vi "Main Page.vi"(8 "error in":errorcluster, 11 "Node Ptr":T1 format="%.0x") -> (0 "error out":errorcluster)   [LabVIEW 2020, in "AIM ARINC 429 System Explorer.lvlib" / "Implementation.lvlib"]
uses:
  Implementation.lvlib
  <vilib>/NI VeriStand/Custom Device API/Custom Device API.lvlib
  Scripting/AIM/AIM ARINC 429 Scripting.lvlib
  <vilib>/NI VeriStand/Custom Device API/Custom Device Item Ref.ctl
panel:
  in  "Coupling Mode":enum32{"External", "Dual", "Internal"}(ring)
  in  "Async Rx Execution":bool
  in  "Decimation":i32=1 min=1
  in  "General Header":cluster{"Section Name":string}={"Section Name"="AIM ARINC 429 - Main"}
  in  "PXI Slot Number":u8=1
  in  "SHDocVw.IWebBrowser":refnum<k7>(container)
  in  "Description":string
  in  "Name":string
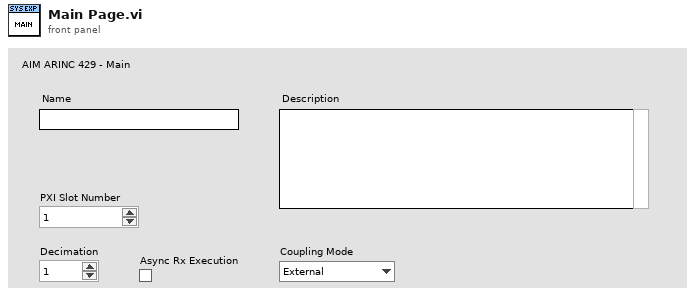
[diagram p1: front panel]
types:
  T1 = typedef "Custom Device API.lvlib/Custom Device Item Ref.ctl" = u64
  T2 = typedef "Device Parameters.ctl" = cluster{"pxi slot":u8, "coupling mode":u32}
  T3 = typedef "Custom Device API.lvlib/Custom Device Item Info.ctl" = cluster{"Name":string, "Is Channel":bool, "GUID":string, "Is Waveform":bool}
  T4 = typedef "Custom Device API.lvlib/Custom Device Commands.ctl" = enum16{"Default", "Item renamed", "Shutdown", "Dynamic button pressed"}
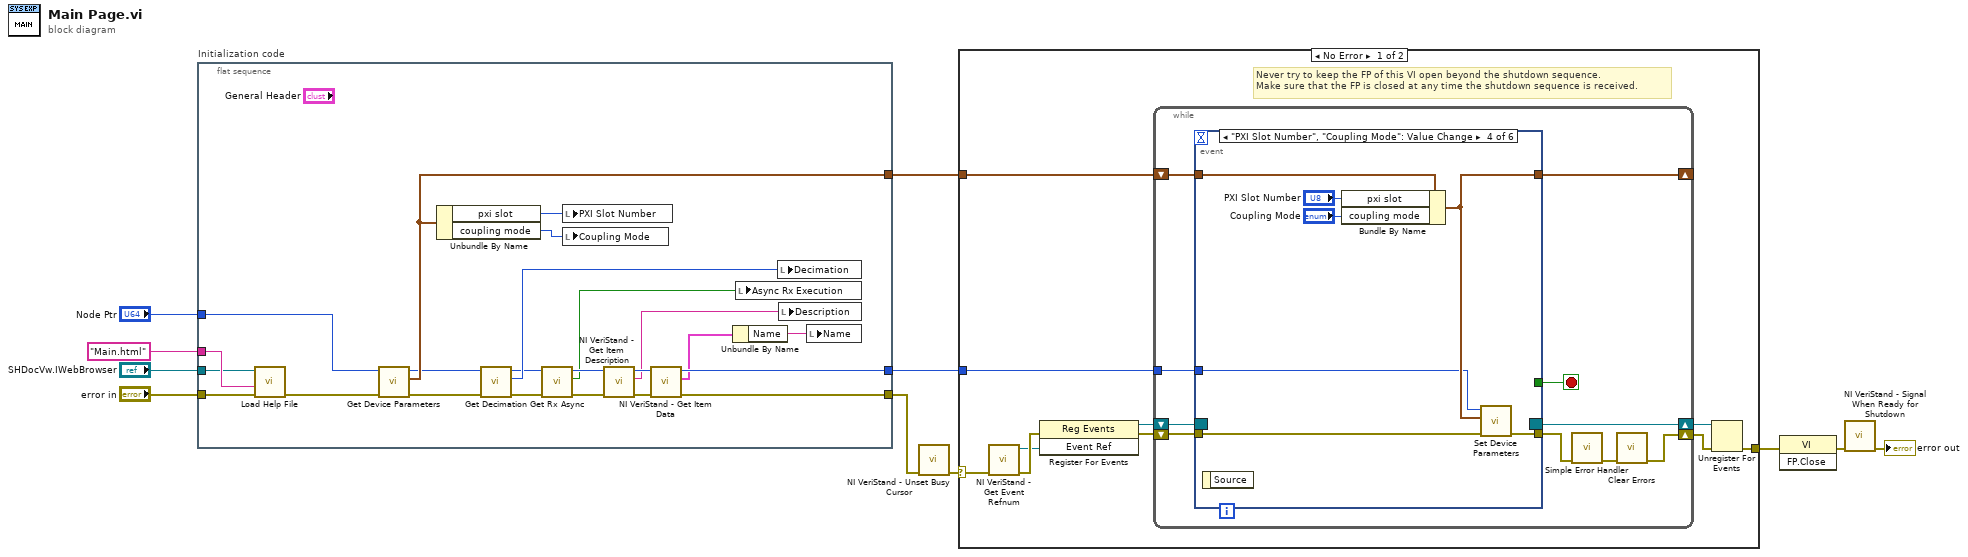
[diagram p0: block diagram]
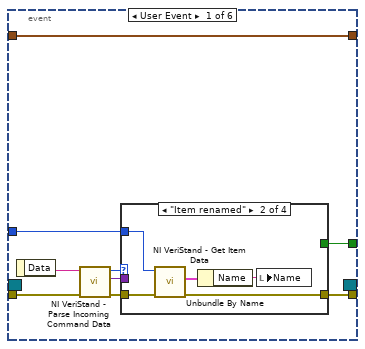
[diagram p2: hidden frame]
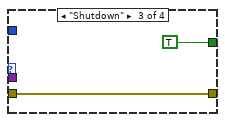
[diagram p4: hidden frame]
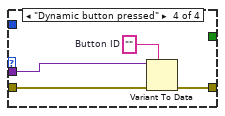
[diagram p5: hidden frame]
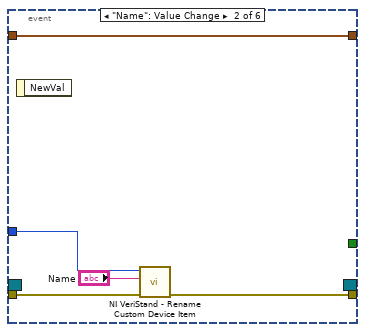
[diagram p6: hidden frame]
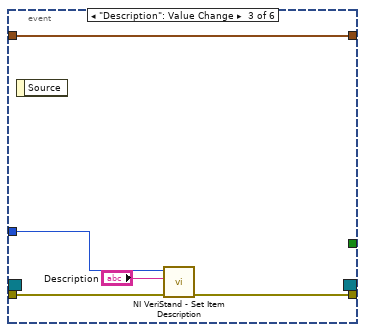
[diagram p7: hidden frame]
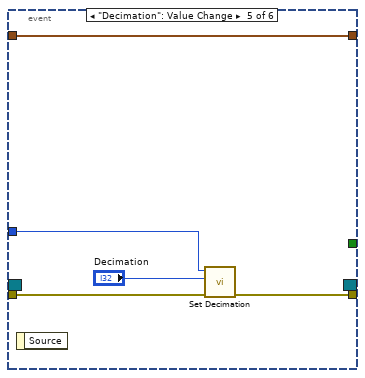
[diagram p8: hidden frame]
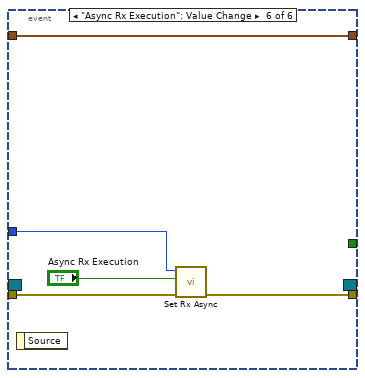
[diagram p9: hidden frame]
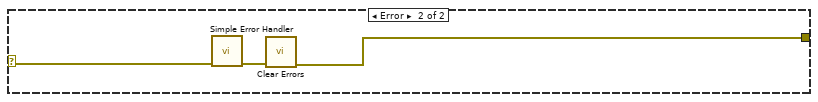
[diagram p10: hidden frame]
diagram:
  n1 = flat-sequence "Initialization code" {
    tunnel: "error in" -> [w27]
    tunnel: "Node Ptr" -> [w23]
    tunnel: [w30] -> w7
    tunnel: [w34] -> w4
    tunnel: "SHDocVw.IWebBrowser" -> [w25]
    tunnel: "Main.html" ("HTML File") -> [w26]
    tunnel: [w22] -> w1
    frame #0 {
      n2 = call "Load Help File.vi"("error in (no error)"=w27, "HTML File to Load"=w26, "Browser"=w25) -> ("error out"=w24:errorcluster)  [unwired: 8 in]
      n3 = call "Get Device Parameters.vi"("error in"=w24, "custom device ref"=w23) -> ("error out"=w21:errorcluster, "device parameters"=w22:T2, "custom device ref out"=w20:T1)  [unwired: 7 in]
      n4 = Unbundle By Name(w22) -> ("pxi slot"=w13:u8, "coupling mode"=w12:u32)
      n5 = call "Get Decimation.vi"("error in"=w21, "custom device ref"=w20) -> ("error out"=w18:errorcluster, "decimation"=w19:i32, "custom device ref out"=w16:T1)  [unwired: 7 in]
      n6 = call "Get Rx Async.vi"("error in"=w18, "custom device ref"=w16) -> ("error out"=w17:errorcluster, "rx async?"=w14:bool, "custom device ref out"=w15:T1)  [unwired: 7 in]
      n7 = local write "PXI Slot Number"(w13) -> ()
      n8 = local write "Coupling Mode"(w12) -> ()
      n9 = call <vilib>:"NI VeriStand - Get Item Description.vi"("error in (no error)"=w17, "Item Ref in"=w15) -> ("error out"=w32:errorcluster, "Description"=w28:string, "Item Ref out"=w33:T1)  [unwired: 7 out]
      n10 = call <vilib>:"NI VeriStand - Get Item Data.vi"("error in (no error)"=w32, "Item Ref in"=w33) -> ("error out"=w30:errorcluster, "Item Info"=w31:T3, "Item Ref out"=w34:T1)  [unwired: 7 out]
      n11 = Unbundle By Name(w31) -> ("Name"=w29:string)
      n12 = local write "Async Rx Execution"(w14) -> ()
      n13 = local write "Decimation"(w19) -> ()
      n14 = local write "Description"(w28) -> ()
      n15 = local write "Name"(w29) -> ()
    }
  }
  n16 = call <vilib>:"NI VeriStand - Unset Busy Cursor.vi"("error in (no error)"=w7) -> ("error out"=w6:errorcluster)  [unwired: 10 out]
  n17 = case shown="No Error" w6 {
    selector: w6 -> [w36 w105]
    tunnel: [w41 w103] -> w11
    tunnel: w4 -> [w37 _]
    tunnel: w1 -> [w35 _]
    frame No Error {
      # "Never try to keep the FP of this VI open beyond the shutdown sequence.\nMake sure that the FP is closed at any time the shutdown sequence is received."
      n18 = call <vilib>:"NI VeriStand - Get Event Refnum.vi"("error in (no error)"=w36) -> ("error out"=w44:errorcluster, "Event Ref"=w40:refnum<user-event>)  [unwired: 9 out]
      n19 = register-events(error in=w44, w40) -> (reference out=w38:refnum<event-registration>, error out=w39:errorcluster)  [unwired: 1 in]
      n20 = while {
        tunnel: w37 -> [w50]
        shift-right: [w47] -> w42
        shift-left: w39 -> [w53]
        shift-right: [w54] -> w43
        shift-left: w38 -> [w52]
        shift-right: [w45] -> _
        shift-left: w35 -> [w46]
        stop <- w51 stop-if-true
        n21 = event shown="[3] \"PXI Slot Number\", \"Coupling Mode\": Value Change" {
          selector: w52 -> [_ _ _ _ _ _]
          dyn-events: [_ _ _ _ _ _] -> w54
          timeout: _ -> [_ _ _ _ _ _]
          tunnel: w53 -> [w63 w80 w84 w90 w96 w101]
          tunnel: [w59 _ _ _ _ _] -> w51
          tunnel: [w58 w79 w83 w89 w95 w99] -> w49
          tunnel: w50 -> [w57 w78 w85 w87 w94 w100]
          tunnel: w46 -> [w55 w76 w81 w92 w97 w102]
          tunnel: [w55 w76 w81 w91 w97 w102] -> w45
          event User Event {
            n22 = event-data() -> ("Data"=w62:string)  [unwired: 1 out]
            n23 = call <vilib>:"NI VeriStand - Parse Incoming Command Data.vi"("error in (no error)"=w63, "Incoming data"=w62) -> ("error out"=w61:errorcluster, "Outgoing data"=w56:variant, "Action"=w60:T4)  [unwired: 7 out]
            n24 = case shown="\"Item renamed\"" w60 {
              tunnel: w61 -> [w64 w69 w70 w75]
              tunnel: [_ _ TRUE _] -> w59
              tunnel: [w64 w66 w70 w72] -> w58
              tunnel: w57 -> [_ w68 _ _]
              tunnel: w56 -> [_ _ _ w74]
              frame "Default", Default {
              }
              frame "Item renamed" {
                n25 = call <vilib>:"NI VeriStand - Get Item Data.vi"("error in (no error)"=w69, "Item Ref in"=w68) -> ("error out"=w66:errorcluster, "Item Info"=w67:T3)  [unwired: 8 out]
                n26 = Unbundle By Name(w67) -> ("Name"=w65:string)
                n27 = local write "Name"(w65) -> ()
              }
              frame "Shutdown" {
              }
              frame "Dynamic button pressed" {
                w73 = ""  # Button ID
                n28 = Variant To Data(error in=w75, type=w73, Variant=w74) -> (error out=w72:errorcluster)  [unwired: 1 out]
              }
            }
          }
          event "Name": Value Change {
            n29 = event-data() -> ()  [unwired: 2 out]
            n30 = call <vilib>:"NI VeriStand - Rename Custom Device Item.vi"("error in (no error)"=w80, "New Name"="Name", "Item Ref in"=w78) -> ("error out"=w79:errorcluster)  [unwired: 1 in, 7 out]
          }
          event "Description": Value Change {
            n31 = event-data() -> ()  [unwired: 2 out]
            n32 = call <vilib>:"NI VeriStand - Set Item Description.vi"("error in (no error)"=w84, "Description"="Description", "Item Ref in"=w85) -> ("error out"=w83:errorcluster)  [unwired: 8 out]
          }
          event "PXI Slot Number", "Coupling Mode": Value Change {
            n33 = event-data() -> ()  [unwired: 2 out]
            n34 = Bundle By Name(cluster=w92, "pxi slot"="PXI Slot Number", "coupling mode"="Coupling Mode") -> (w91:T2)
            n35 = call "Set Device Parameters.vi"("error in"=w90, "device parameters"=w91, "custom device"=w87) -> ("error out"=w89:errorcluster)  [unwired: 7 in, 1 out]
          }
          event "Decimation": Value Change {
            n36 = event-data() -> ()  [unwired: 2 out]
            n37 = call "Set Decimation.vi"("error in"=w96, "decimation"="Decimation", "custom device ref"=w94) -> ("error out"=w95:errorcluster)  [unwired: 7 in, 1 out]
          }
          event "Async Rx Execution": Value Change {
            n38 = event-data() -> ()  [unwired: 2 out]
            n39 = call "Set Rx Async.vi"("error in"=w101, "rx async?"="Async Rx Execution", "custom device ref"=w100) -> ("error out"=w99:errorcluster)  [unwired: 7 in, 1 out]
          }
        }
        n40 = call <vilib>:"Simple Error Handler.vi"("error in (no error)"=w49) -> ("error out"=w48:errorcluster)  [unwired: 1 in, 7 out]
        n41 = call <vilib>:"Clear Errors.vi"("error in (no error)"=w48) -> ("error out"=w47:errorcluster)  [unwired: 1 in, 5 out]
      }
      n42 = Unregister For Events(event registration refnum=w43, error in=w42) -> (error out=w41:errorcluster)
    }
    frame Error {
      n43 = call <vilib>:"Simple Error Handler.vi"("error in (no error)"=w105) -> ("error out"=w104:errorcluster)  [unwired: 1 in, 7 out]
      n44 = call <vilib>:"Clear Errors.vi"("error in (no error)"=w104) -> ("error out"=w103:errorcluster)  [unwired: 1 in, 5 out]
    }
  }
  n45 = invoke class="VI" method="FP.Close"(error in=w11) -> (error out=w10:errorcluster)  [unwired: 2 in, 2 out]
  n46 = call <vilib>:"NI VeriStand - Signal When Ready for Shutdown.vi"("error in (no error)"=w10) -> ("error out"=→"error out":errorcluster)  [unwired: 10 out]
